vi "non-overlap.vi"(8 "error in":errorcluster, 11 "String":string) -> (0 "error out":errorcluster, 2 "Array 3":cluster{string, bool}[](array[cluster]), 3 "non-overlapped array":string[](array[string]))   [LabVIEW 2018]
panel:
  out "Array 4":string[](array[string])
  out "Array 2":string[](array[string])
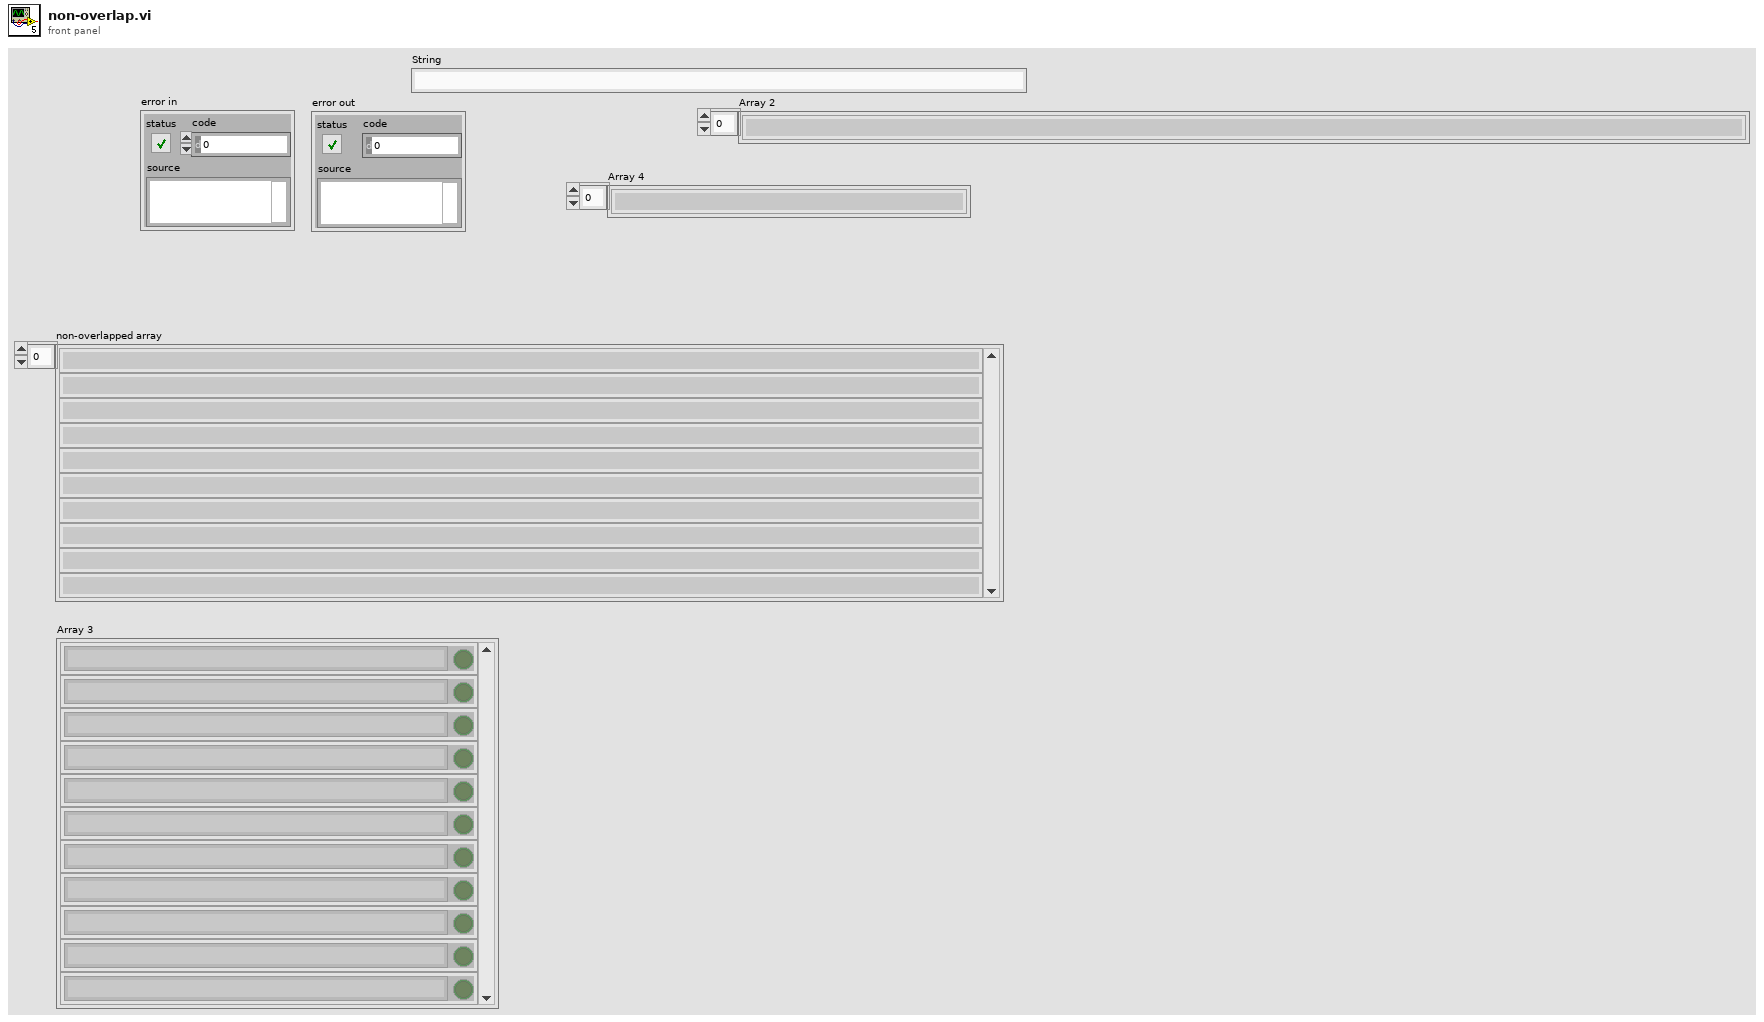
[diagram p1: front panel]
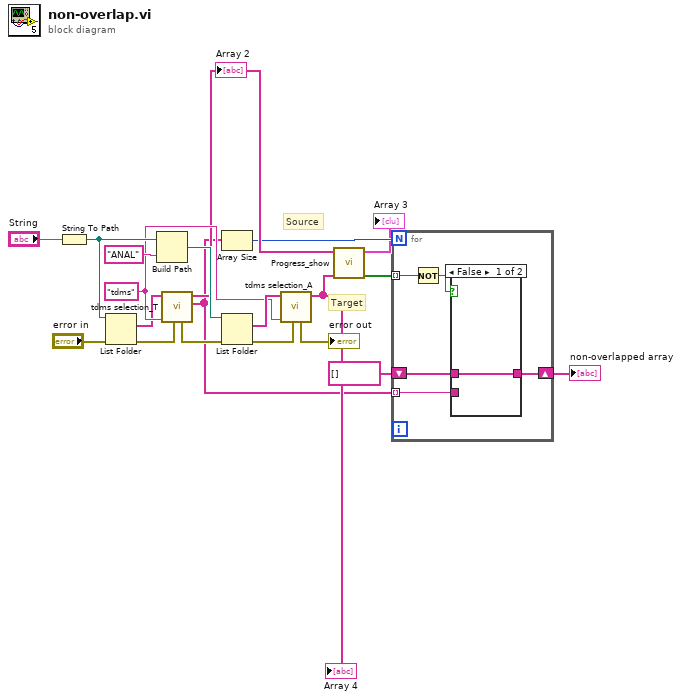
[diagram p0: block diagram]
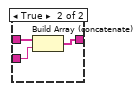
[diagram p2: hidden frame]
diagram:
  w10 = "tdms" ("string")
  # "Target"
  # "Source"
  n1 = String To Path(string="String") -> (path=w16:path)
  n2 = List Folder(path=w16, error in="error in") -> (filenames=w9:string[], error out=w13:errorcluster)  [unwired: 2 in, 2 out]
  n3 = Build Path(base path=w16, name or relative path="ANAL" ("文字列")) -> (appended path=w17:path)
  n4 = call "tdms selection_T.vi"("error in"=w13, "string"=w10, "Filename List"=w9) -> ("Array"=w4:string[], "Array 2"=w6:string[], "error out"=w12:errorcluster)  [unwired: 5 in, 1 out]
  "Array 2" <- w6
  n5 = Array Size(array=w4) -> (size(s)=w5:i32)
  n6 = List Folder(path=w17, error in=w12) -> (filenames=w11:string[], error out=w8:errorcluster)  [unwired: 2 in, 2 out]
  n7 = call "tdms selection_A.vi"("error in"=w8, "string"=w10, "Filename List"=w11) -> ("Array 2"=w7:string[], "error out"=→"error out":errorcluster)  [unwired: 6 in, 1 out]
  "Array 4" <- w7
  n8 = call "Progress_show.vi"("P_folder names"=w7, "folder names"=w6) -> ("Array"=w15:bool[], "Array 3"=→"Array 3":cluster{string, bool}[])  [unwired: 6 in, 2 out]
  n9 = for {
    N: w5 -> [_]
    tunnel: w15 -> [w25] mode=indexing
    shift-right: [w22] -> w14
    shift-left: string[] [] -> [w24]
    tunnel: w4 -> [w23] mode=indexing
    n10 = Not(x=w25) -> (.not. x?=w21:bool)
    n11 = case shown="False" w21 {
      tunnel: [w26 w29] -> w22
      tunnel: w24 -> [w26 w28]
      tunnel: w23 -> [_ w27]
      frame False {
      }
      frame True {
        n12 = Build Array (concatenate)(w28, w27) -> (w29:string[])
      }
    }
  }
  "non-overlapped array" <- w14
